vi "扫雷.vi"() -> ()   [LabVIEW 2017]
panel:
  out "上次索引":i32
  out "地图":u16[][](array[ring])
  out "游戏进行中":bool
  out "花费时间":dbl format="%<%M:%S>t"
  out "剩余地雷数":i32
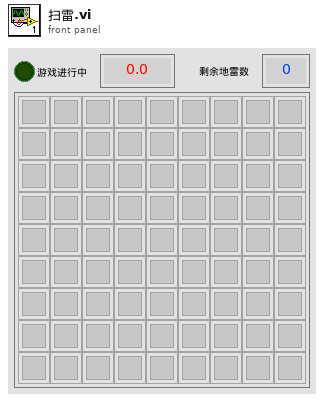
[diagram p1: front panel]
types:
  T1 = enum8{"Enabled", "Disabled", "Disabled and Grayed Out"}
  T2 = typedef "LVRectTypeDef.ctl" = cluster{"Left":i16, "Top":i16, "Right":i16, "Bottom":i16}
  T3 = typedef "LVBoundsTypeDef.ctl" = cluster{"Width":u32, "Height":u32}
  T4 = typedef "LVPositionTypeDef.ctl" = cluster{"Left":i32, "Top":i32}
  T5 = typedef "LVPoint32TypeDef.ctl" = cluster{"Horizontal":i32, "Vertical":i32}
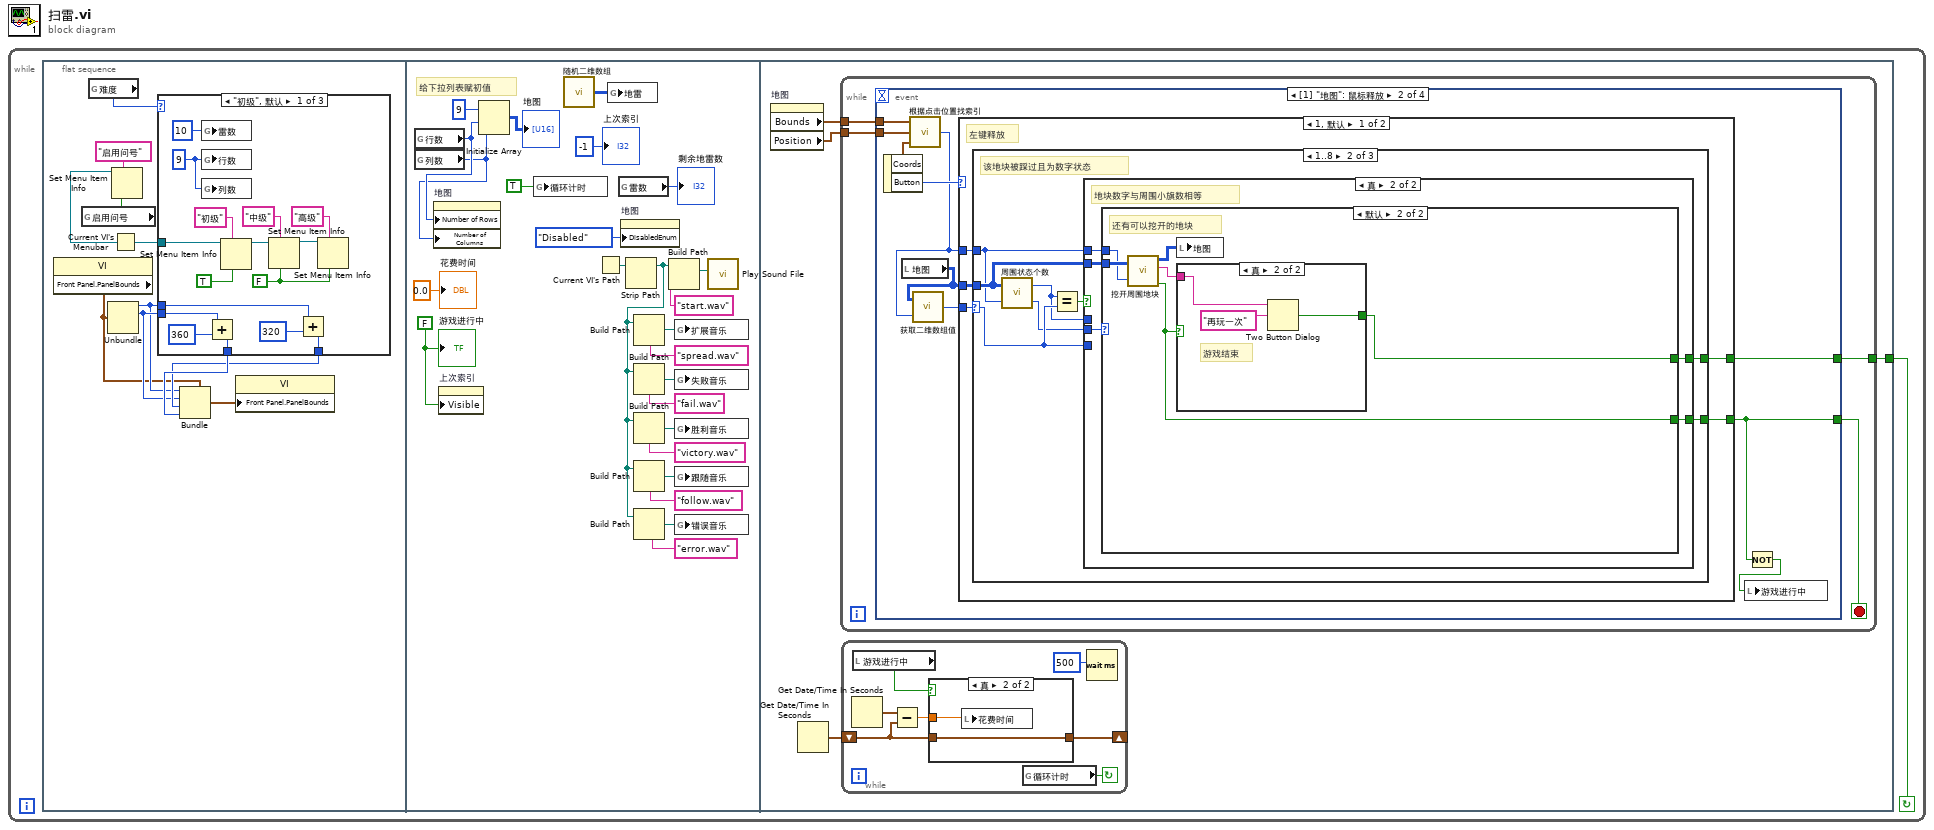
[diagram p0: block diagram]
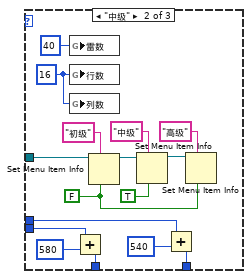
[diagram p2: hidden frame]
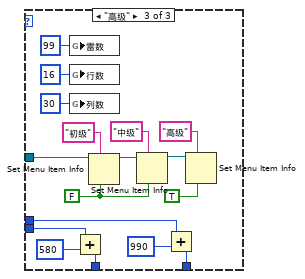
[diagram p3: hidden frame]
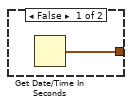
[diagram p4: hidden frame]
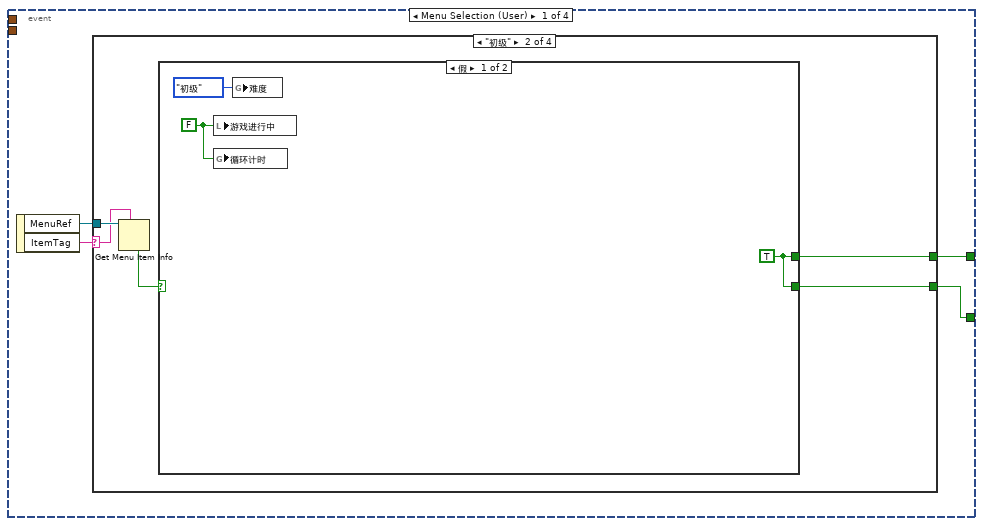
[diagram p5: hidden frame]
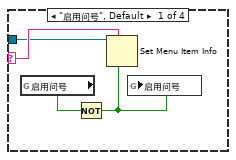
[diagram p6: hidden frame]
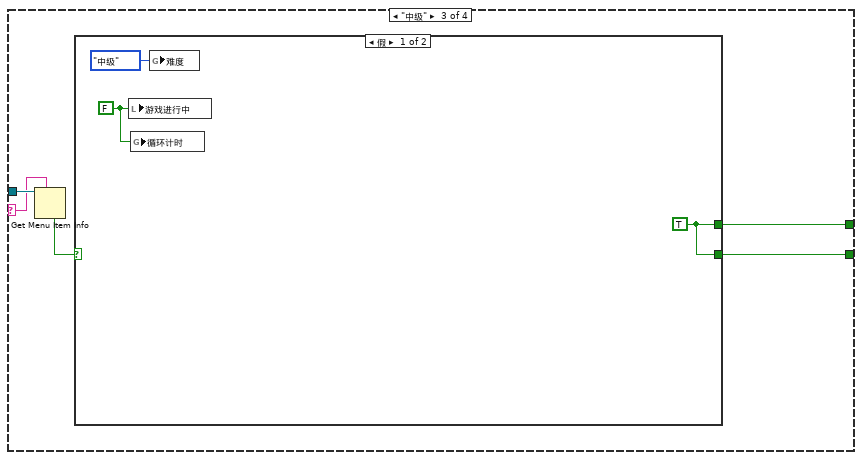
[diagram p8: hidden frame]
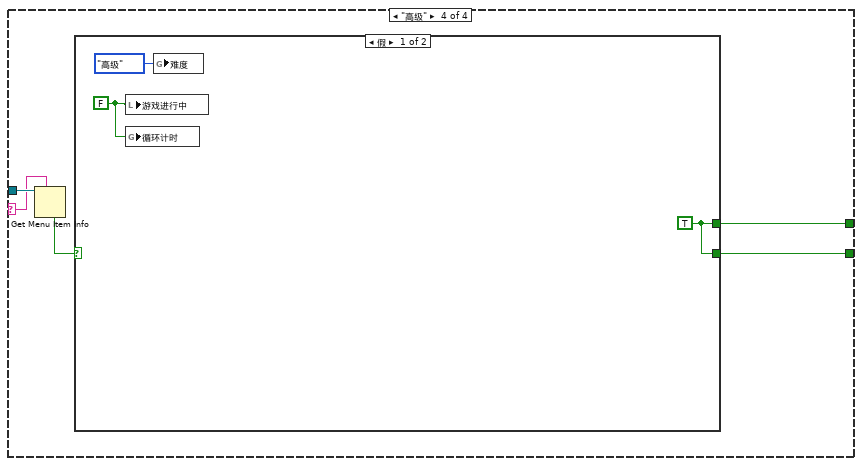
[diagram p10: hidden frame]
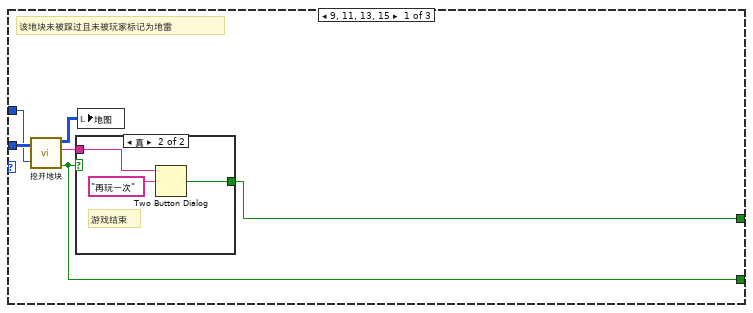
[diagram p12: hidden frame]
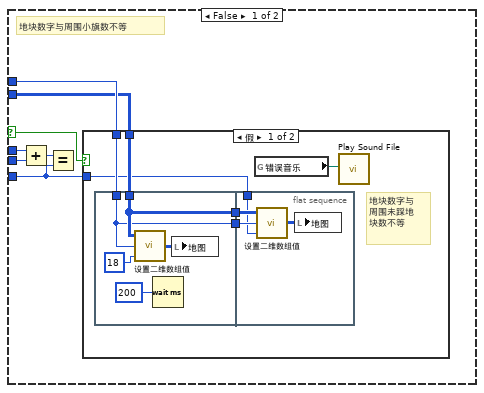
[diagram p14: hidden frame]
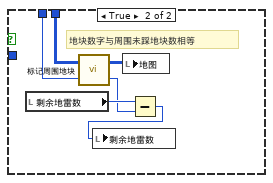
[diagram p15: hidden frame]
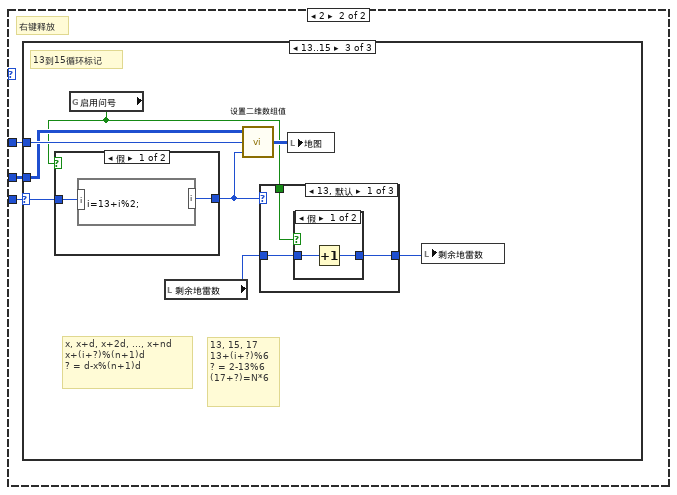
[diagram p19: hidden frame]
diagram:
  n1 = while {
    stop <- w1 continue-if-true
    n2 = flat-sequence {
      tunnel: [w89] -> w1
      frame #0 {
        n3 = property class="VI"() -> ("Front Panel.PanelBounds"=w2:T2)  [unwired: 2 in, 2 out]
        n4 = global read "全局变量.vi" "启用问号"() -> (w8:bool)
        n5 = global read "全局变量.vi" "难度"() -> (w11:enum16{"初级", "中级", "高级"})
        n6 = Unbundle(w2) -> ("Left"=w4:i16, "Top"=w5:i16)  [unwired: 2 out]
        n7 = Current VI's Menubar() -> (w9:refnum<k9>)
        n8 = Set Menu Item Info(6:w8, 7:"启用问号" ("项标识符"), 11:w9) -> ()  [unwired: 4 in, 2 out]
        n9 = case shown="\"初级\", 默认" w11 {
          tunnel: w9 -> [w18 w34 w50]
          tunnel: w4 -> [w17 w31 w47]
          tunnel: w5 -> [w16 w30 w46]
          tunnel: [w13 w28 w44] -> w6
          tunnel: [w15 w29 w45] -> w7
          frame "初级", Default {
            w19 = FALSE ("已勾选")
            w27 = i16 9 ("雷数")
            n10 = global write "全局变量.vi" "雷数"(i16 10 ("雷数")) -> ()
            n11 = global write "全局变量.vi" "行数"(w27) -> ()
            n12 = global write "全局变量.vi" "列数"(w27) -> ()
            n13 = Add(x=w16, y=i16 360) -> (x+y=w15:i16)
            n14 = Set Menu Item Info(6:TRUE ("已勾选"), 7:"初级" ("项标识符"), 11:w18) -> (3:w25:refnum<k9>)  [unwired: 4 in, 1 out]
            n15 = Set Menu Item Info(6:w19, 7:"中级" ("项标识符"), 11:w25) -> (3:w24:refnum<k9>)  [unwired: 4 in, 1 out]
            n16 = Add(x=w17, y=i16 320) -> (x+y=w13:i16)
            n17 = Set Menu Item Info(6:w19, 7:"高级" ("项标识符"), 11:w24) -> ()  [unwired: 4 in, 2 out]
          }
          frame "中级" {
            w35 = FALSE ("已勾选")
            w43 = i16 16 ("雷数")
            n18 = global write "全局变量.vi" "雷数"(i16 40 ("雷数")) -> ()
            n19 = global write "全局变量.vi" "行数"(w43) -> ()
            n20 = global write "全局变量.vi" "列数"(w43) -> ()
            n21 = Add(x=w30, y=i16 580) -> (x+y=w29:i16)
            n22 = Set Menu Item Info(6:w35, 7:"初级" ("项标识符"), 11:w34) -> (3:w41:refnum<k9>)  [unwired: 4 in, 1 out]
            n23 = Set Menu Item Info(6:TRUE ("已勾选"), 7:"中级" ("项标识符"), 11:w41) -> (3:w40:refnum<k9>)  [unwired: 4 in, 1 out]
            n24 = Add(x=w31, y=i16 540) -> (x+y=w28:i16)
            n25 = Set Menu Item Info(6:w35, 7:"高级" ("项标识符"), 11:w40) -> ()  [unwired: 4 in, 2 out]
          }
          frame "高级" {
            w51 = FALSE ("已勾选")
            n26 = global write "全局变量.vi" "雷数"(i16 99 ("雷数")) -> ()
            n27 = global write "全局变量.vi" "行数"(i16 16 ("雷数")) -> ()
            n28 = global write "全局变量.vi" "列数"(i16 30 ("列数")) -> ()
            n29 = Add(x=w46, y=i16 580) -> (x+y=w45:i16)
            n30 = Set Menu Item Info(6:w51, 7:"初级" ("项标识符"), 11:w50) -> (3:w57:refnum<k9>)  [unwired: 4 in, 1 out]
            n31 = Set Menu Item Info(6:w51, 7:"中级" ("项标识符"), 11:w57) -> (3:w56:refnum<k9>)  [unwired: 4 in, 1 out]
            n32 = Add(x=w47, y=i16 990) -> (x+y=w44:i16)
            n33 = Set Menu Item Info(6:TRUE ("已勾选"), 7:"高级" ("项标识符"), 11:w56) -> ()  [unwired: 4 in, 2 out]
          }
        }
        n34 = Bundle(cluster=w2, "Left"=w4, "Top"=w5, "Right"=w6, "Bottom"=w7) -> (w3:T2)
        n35 = property class="VI"("Front Panel.PanelBounds"=w3) -> ()  [unwired: 2 in, 2 out]
      }
      frame #1 {
        w72 = FALSE ("游戏进行中")
        # "给下拉列表赋初值"
        n36 = global read "全局变量.vi" "行数"() -> (w62:i32)
        n37 = global read "全局变量.vi" "列数"() -> (w61:i32)
        n38 = property on="地图" class="Arr (严格)"("Number of Rows"=w62, "Number of Columns"=w61) -> ()  [unwired: 2 in, 2 out]
        n39 = property on="上次索引" class="DigNum (严格)"("Visible"=w72) -> ()  [unwired: 2 in, 2 out]
        n40 = Initialize Array(9, w62, w61) -> (→"地图":i32[][])
        n41 = global write "全局变量.vi" "循环计时"(TRUE ("计时循环")) -> ()
        n42 = call "随机二维数组.vi"() -> ("数组"=w85:i16[][])
        n43 = Current VI's Path() -> (path=w81:path)
        n44 = global write "全局变量.vi" "地雷"(w85) -> ()
        n45 = global read "全局变量.vi" "雷数"() -> (→"剩余地雷数":i32)
        n46 = property on="地图" class="Arr (严格)"("DisabledEnum"=T1."Disabled" ("禁用")) -> ()  [unwired: 2 in, 2 out]
        n47 = Strip Path(path=w81) -> (stripped path=w74:path)  [unwired: 1 out]
        n48 = Build Path(base path=w74, name or relative path="spread.wav" ("名称或相对路径")) -> (appended path=w71:path)
        n49 = Build Path(base path=w74, name or relative path="fail.wav" ("名称或相对路径")) -> (appended path=w70:path)
        n50 = Build Path(base path=w74, name or relative path="victory.wav" ("名称或相对路径")) -> (appended path=w69:path)
        n51 = Build Path(base path=w74, name or relative path="follow.wav" ("名称或相对路径")) -> (appended path=w68:path)
        n52 = Build Path(base path=w74, name or relative path="error.wav" ("名称或相对路径")) -> (appended path=w67:path)
        n53 = Build Path(base path=w74, name or relative path="start.wav" ("名称或相对路径")) -> (appended path=w80:path)
        n54 = global write "全局变量.vi" "扩展音乐"(w71) -> ()
        n55 = global write "全局变量.vi" "失败音乐"(w70) -> ()
        n56 = global write "全局变量.vi" "胜利音乐"(w69) -> ()
        n57 = global write "全局变量.vi" "跟随音乐"(w68) -> ()
        n58 = global write "全局变量.vi" "错误音乐"(w67) -> ()
        n59 = call <vilib>:"Play Sound File.vi"("path"=w80) -> ()  [unwired: 9 in, 2 out]
        "游戏进行中" <- w72
        "花费时间" <- 0.0 ("花费时间")
        "上次索引" <- -1 ("上次索引")
      }
      frame #2 {
        n60 = property on="地图" class="Arr (严格)"() -> ("Bounds"=w87:T3, "Position"=w86:T4)  [unwired: 2 in, 2 out]
        n61 = Get Date/Time In Seconds() -> (seconds since 1Jan1904=w88:timestamp)
        n62 = while {
          tunnel: [w101] -> w89
          tunnel: w87 -> [w103]
          tunnel: w86 -> [w102]
          stop <- w100 stop-if-true
          n63 = event shown="[1] \"地图\": 鼠标释放" {
            selector: _ -> [_ _ _ _]
            dyn-events: _ -> [_ _ _ _]
            timeout: _ -> [_ _ _ _]
            tunnel: [w105 w141 _ _] -> w101
            tunnel: w103 -> [_ w145 w240 _]
            tunnel: w102 -> [_ w144 w239 _]
            tunnel: [w104 w140 _ _] -> w100
            event Menu Selection (User) {
              n64 = event-data() -> ("MenuRef"=w106:refnum<k9>, "ItemTag"=w107:string)  [unwired: 1 in]
              n65 = case shown="\"初级\"" w107 {
                selector: w107 -> [w111 w114 w122 w130]
                tunnel: w106 -> [w109 w116 w123 w131]
                tunnel: [_ w113 w121 w129] -> w105
                tunnel: [_ w112 w120 w128] -> w104
                frame "启用问号", Default {
                  n66 = global read "全局变量.vi" "启用问号"() -> (w110:bool)
                  n67 = Not(x=w110) -> (.not. x?=w108:bool)
                  n68 = Set Menu Item Info(6:w108, 7:w111, 11:w109) -> ()  [unwired: 4 in, 2 out]
                  n69 = global write "全局变量.vi" "启用问号"(w108) -> ()
                }
                frame "初级" {
                  n70 = Get Menu Item Info(7:w114, 11:w116) -> (4:w115:bool)  [unwired: 1 in, 6 out]
                  n71 = case shown="假" w115 {
                    tunnel: [w119 _] -> w113
                    tunnel: [w119 _] -> w112
                    frame False {
                      w118 = FALSE ("游戏进行中")
                      w119 = TRUE
                      n72 = local write "游戏进行中"(w118) -> ()
                      n73 = global write "全局变量.vi" "循环计时"(w118) -> ()
                      n74 = global write "全局变量.vi" "难度"(enum16{"初级", "中级", "高级"}."初级" ("难度")) -> ()
                    }
                    frame True {
                    }
                  }
                }
                frame "中级" {
                  n75 = Get Menu Item Info(7:w122, 11:w123) -> (4:w124:bool)  [unwired: 1 in, 6 out]
                  n76 = case shown="假" w124 {
                    tunnel: [w127 _] -> w121
                    tunnel: [w127 _] -> w120
                    frame False {
                      w125 = FALSE ("游戏进行中")
                      w127 = TRUE
                      n77 = local write "游戏进行中"(w125) -> ()
                      n78 = global write "全局变量.vi" "循环计时"(w125) -> ()
                      n79 = global write "全局变量.vi" "难度"(enum16{"初级", "中级", "高级"}."中级" ("难度")) -> ()
                    }
                    frame True {
                    }
                  }
                }
                frame "高级" {
                  n80 = Get Menu Item Info(7:w130, 11:w131) -> (4:w132:bool)  [unwired: 1 in, 6 out]
                  n81 = case shown="假" w132 {
                    tunnel: [w135 _] -> w129
                    tunnel: [w135 _] -> w128
                    frame False {
                      w133 = FALSE ("游戏进行中")
                      w135 = TRUE
                      n82 = local write "游戏进行中"(w133) -> ()
                      n83 = global write "全局变量.vi" "循环计时"(w133) -> ()
                      n84 = global write "全局变量.vi" "难度"(enum16{"初级", "中级", "高级"}."高级" ("难度")) -> ()
                    }
                    frame True {
                    }
                  }
                }
              }
            }
            event "地图": Mouse Up {
              n85 = event-data() -> ("Coords"=w143:T5, "Button"=w142:u16)  [unwired: 1 in]
              n86 = local read "地图"() -> (w137:u16[][])
              n87 = call "根据点击位置找索引.vi"("坐标"=w143, "位置"=w144, "边界"=w145) -> ("索引"=w138:i32)
              n88 = call "获取二维数组值.vi"("索引"=w138, "数组"=w137) -> ("数值"=w139:i32)
              n89 = case shown="1, 默认" w142 {
                tunnel: [w150 _] -> w141
                tunnel: [w149 _] -> w140
                tunnel: w139 -> [w148 w212]
                tunnel: w138 -> [w147 w211]
                tunnel: w137 -> [w146 w210]
                frame 1, Default {
                  # "左键释放"
                  n90 = case shown="1..8" w148 {
                    selector: w148 -> [_ w166 _]
                    tunnel: [w151 w161 _] -> w150
                    tunnel: [w153 w160 _] -> w149
                    tunnel: w147 -> [w155 w164 _]
                    tunnel: w146 -> [w156 w165 _]
                    frame 9, 11, 13, 15 {
                      # "该地块未被踩过且未被玩家标记为地雷"
                      n91 = call "挖开地块.vi"("地图"=w156, "索引"=w155) -> ("输出地图"=w154:i32[][], "对话框信息"=w152:string, "游戏结束"=w153:bool)  [unwired: 1 out]
                      n92 = case shown="真" w153 {
                        tunnel: w152 -> [_ w158]
                        tunnel: [_ w157] -> w151
                        frame False {
                        }
                        frame True {
                          # "游戏结束"
                          n93 = Two Button Dialog(message=w158, 2:"再玩一次" ("T按钮名称（“确定”）")) -> (T button?=w157:bool)  [unwired: 1 in]
                        }
                      }
                      n94 = local write "地图"(w154) -> ()
                    }
                    frame 1..8 {
                      # "该地块被踩过且为数字状态"
                      n95 = call "周围状态个数.vi"("索引"=w164, "地图"=w165) -> ("未标记数"=w162:i32, "标记数"=w163:i32)
                      n96 = Equal?(x=w163, y=w166) -> (x = y?=w167:bool)
                      n97 = case shown="真" w167 {
                        selector: w167 -> [w168 _]
                        tunnel: w165 -> [w172 w199]
                        tunnel: w164 -> [w173 w198]
                        tunnel: w166 -> [w171 _]
                        tunnel: w163 -> [w170 _]
                        tunnel: w162 -> [w169 w200]
                        tunnel: [_ w197] -> w161
                        tunnel: [_ w196] -> w160
                        frame False {
                          # "地块数字与周围小旗数不等"
                          n98 = Add(x=w170, y=w169) -> (x+y=w174:i32)
                          n99 = Equal?(x=w174, y=w171) -> ()  [unwired: 1 out]
                          n100 = case shown="假" w168 {
                            tunnel: w173 -> [w179 w195]
                            tunnel: w172 -> [w180 w194]
                            tunnel: w171 -> [w176 _]
                            frame False {
                              # "地块数字与\n周围未踩地\n块数不等"
                              n101 = flat-sequence {
                                tunnel: w180 -> [w183]
                                tunnel: w179 -> [w182]
                                tunnel: [w183] -> w178
                                tunnel: [w182] -> w177
                                tunnel: w178 -> [w189]
                                tunnel: w177 -> [w188]
                                tunnel: w176 -> [w187]
                                frame #0 {
                                n102 = call "设置二维数组值.vi"("数值"=18, "索引"=w182, "数组"=w183) -> ("输出数组"=w184:i32[][])
                                n103 = Wait (ms)(milliseconds to wait=u32 200 ("毫秒倍数")) -> ()  [unwired: 1 out]
                                n104 = local write "地图"(w184) -> ()
                                }
                                frame #1 {
                                n105 = call "设置二维数组值.vi"("数值"=w187, "索引"=w188, "数组"=w189) -> ("输出数组"=w186:i32[][])
                                n106 = local write "地图"(w186) -> ()
                                }
                              }
                              n107 = global read "全局变量.vi" "错误音乐"() -> (w175:path)
                              n108 = call <vilib>:"Play Sound File.vi"("path"=w175) -> ()  [unwired: 9 in, 2 out]
                            }
                            frame True {
                              # "地块数字与周围未踩地块数相等"
                              n109 = local read "剩余地雷数"() -> (w192:i32)
                              n110 = call "标记周围地块.vi"("索引"=w195, "地图"=w194) -> ("标记个数"=w191:i32, "输出地图"=w193:i32[][])
                              n111 = local write "地图"(w193) -> ()
                              n112 = Subtract(x=w192, y=w191) -> (x-y=w190:i32)
                              n113 = local write "剩余地雷数"(w190) -> ()
                            }
                          }
                        }
                        frame True {
                          # "地块数字与周围小旗数相等"
                          n114 = case shown="默认" w200 {
                            tunnel: w199 -> [_ w206]
                            tunnel: w198 -> [_ w205]
                            tunnel: [_ w202] -> w197
                            tunnel: [_ w201] -> w196
                            frame 0 {
                              # "没有可以挖开的地块"
                            }
                            frame Default {
                              # "还有可以挖开的地块"
                              n115 = call "挖开周围地块.vi"("地图"=w206, "索引"=w205) -> ("输出地图"=w204:i32[][], "对话框信息"=w203:string, "游戏结束"=w201:bool)  [unwired: 1 out]
                              n116 = local write "地图"(w204) -> ()
                              n117 = case shown="真" w201 {
                                tunnel: w203 -> [_ w208]
                                tunnel: [_ w207] -> w202
                                frame False {
                                }
                                frame True {
                                # "游戏结束"
                                n118 = Two Button Dialog(message=w208, 2:"再玩一次" ("T按钮名称（“确定”）")) -> (T button?=w207:bool)  [unwired: 1 in]
                                }
                              }
                            }
                          }
                        }
                      }
                    }
                    frame 10, 14, Default {
                      # "该地块被玩家标记为地雷"
                    }
                  }
                }
                frame 2 {
                  # "右键释放"
                  n119 = case shown="13..15" w212 {
                    selector: w212 -> [_ _ w218]
                    tunnel: w211 -> [_ _ w220]
                    tunnel: w210 -> [_ _ w214]
                    frame Default {
                      # "无响应"
                    }
                    frame 1..8 {
                      # "地块为数字状态"
                    }
                    frame 13..15 {
                      # "13, 15, 17\n13+(i+?)%6\n? = 2-13%6\n(17+?)=N*6"
                      # "x, x+d, x+2d, ..., x+nd\nx+(i+?)%(n+1)d\n? = d-x%(n+1)d"
                      # "13到15循环标记"
                      n120 = global read "全局变量.vi" "启用问号"() -> (w213:bool)
                      n121 = case shown="假" w213 {
                        tunnel: w218 -> [w222 w224]
                        tunnel: [w221 w223] -> w217
                        frame False {
                          n122 = formula code="i=13+i%2;"("i"=w222) -> ("i"=w221:i32)
                        }
                        frame True {
                          n123 = formula code="i=13+i%3;"("i"=w224) -> ("i"=w223:i32)
                        }
                      }
                      n124 = local read "剩余地雷数"() -> (w215:i32)
                      n125 = call "设置二维数组值.vi"("数值"=w217, "索引"=w220, "数组"=w214) -> ("输出数组"=w219:i32[][])
                      n126 = case shown="13, 默认" w217 {
                        tunnel: [w226 w231 w233] -> w216
                        tunnel: w215 -> [w227 w232 w234]
                        tunnel: w213 -> [w225 _ _]
                        frame 13, Default {
                          n127 = case shown="假" w225 {
                            tunnel: w227 -> [w229 w230]
                            tunnel: [w228 w230] -> w226
                            frame False {
                              n128 = Increment(x=w229) -> (x+1=w228:i32)
                            }
                            frame True {
                            }
                          }
                        }
                        frame 14 {
                          n129 = Decrement(x=w232) -> (x-1=w231:i32)
                        }
                        frame 15 {
                          n130 = Increment(x=w234) -> (x+1=w233:i32)
                        }
                      }
                      n131 = local write "地图"(w219) -> ()
                      n132 = local write "剩余地雷数"(w216) -> ()
                    }
                  }
                }
              }
              n133 = Not(x=w140) -> (.not. x?=w136:bool)
              n134 = local write "游戏进行中"(w136) -> ()
            }
            event "地图": Mouse Move {
              n135 = event-data() -> ("Coords"=w238:T5)  [unwired: 1 in]
              n136 = call "根据点击位置找索引.vi"("坐标"=w238, "位置"=w239, "边界"=w240) -> ("索引"=w235:i32)
              n137 = local read "地图"() -> (w236:u16[][])
              n138 = call "获取二维数组值.vi"("索引"=w235, "数组"=w236) -> ("数值"=w237:i32)
              n139 = case shown="9..11" w237 {
                selector: w237 -> [_ w255 _]
                tunnel: w236 -> [w241 w256 _]
                tunnel: w235 -> [_ w254 _]
                frame 0..8 {
                  # "当前地块为数字状态"
                  n140 = local read "上次索引"() -> (w242:i32)
                  n141 = case shown="0, 默认" w242 {
                    selector: w242 -> [_ w244]
                    tunnel: w241 -> [_ w243]
                    frame -1 {
                    }
                    frame 0, Default {
                      n142 = call "获取二维数组值.vi"("索引"=w244, "数组"=w243) -> ("数值"=w245:i32)
                      n143 = case shown="13..15" w245 {
                        selector: w245 -> [_ w250]
                        tunnel: w244 -> [_ w252]
                        tunnel: w243 -> [_ w251]
                        frame 0, Default {
                        }
                        frame 13..15 {
                          n144 = Subtract(x=w250, y=4) -> (x-y=w249:i32)
                          n145 = call "设置二维数组值.vi"("数值"=w249, "索引"=w252, "数组"=w251) -> ("输出数组"=w247:i32[][])
                          n146 = local write "上次索引"(-1 ("上次索引")) -> ()
                          n147 = local write "地图"(w247) -> ()
                        }
                      }
                    }
                  }
                }
                frame 9..11 {
                  # "当前地块为初始状态"
                  n148 = flat-sequence {
                    tunnel: w256 -> [w265]
                    tunnel: w255 -> [w264]
                    tunnel: w254 -> [w258]
                    tunnel: [w258] -> w253
                    tunnel: w253 -> [w278]
                    frame #0 {
                      n149 = local read "上次索引"() -> (w259:i32)
                      n150 = Add(x=w264, y=4) -> (x+y=w263:i32)
                      n151 = call "设置二维数组值.vi"("数值"=w263, "索引"=w258, "数组"=w265) -> ("输出数组"=w261:i32[][])
                      n152 = case shown="0, 默认" w259 {
                        selector: w259 -> [_ w269]
                        tunnel: w261 -> [w266 w270]
                        tunnel: [w266 w268] -> w260
                        frame -1 {
                        }
                        frame 0, Default {
                          n153 = call "获取二维数组值.vi"("索引"=w269, "数组"=w270) -> ("数值"=w267:i32)
                          n154 = case shown="13..15" w267 {
                            selector: w267 -> [_ w272]
                            tunnel: w270 -> [w271 w275]
                            tunnel: w269 -> [_ w274]
                            tunnel: [w271 w273] -> w268
                            frame 0, Default {
                            }
                            frame 13..15 {
                              n155 = Subtract(x=w272, y=4) -> (x-y=w276:i32)
                              n156 = call "设置二维数组值.vi"("数值"=w276, "索引"=w274, "数组"=w275) -> ("输出数组"=w273:i32[][])
                            }
                          }
                        }
                      }
                      n157 = global read "全局变量.vi" "跟随音乐"() -> (w257:path)
                      n158 = call <vilib>:"Play Sound File.vi"("path"=w257) -> ()  [unwired: 9 in, 2 out]
                      n159 = local write "地图"(w260) -> ()
                    }
                    frame #1 {
                      n160 = local write "上次索引"(w278) -> ()
                    }
                  }
                }
                frame 13..15, Default {
                  # "当前地块为鼠标跟随状态"
                }
              }
            }
            event "地图": Mouse Leave {
              n161 = event-data() -> ()  [unwired: 1 in, 4 out]
              n162 = local read "上次索引"() -> (w279:i32)
              n163 = case shown="0, 默认" w279 {
                selector: w279 -> [_ w281]
                frame -1 {
                }
                frame 0, Default {
                  n164 = local read "地图"() -> (w280:u16[][])
                  n165 = call "获取二维数组值.vi"("索引"=w281, "数组"=w280) -> ("数值"=w282:i32)
                  n166 = case shown="13..15" w282 {
                    selector: w282 -> [_ w287]
                    tunnel: w281 -> [_ w289]
                    tunnel: w280 -> [_ w288]
                    frame 0, Default {
                    }
                    frame 13..15 {
                      n167 = Subtract(x=w287, y=4) -> (x-y=w286:i32)
                      n168 = call "设置二维数组值.vi"("数值"=w286, "索引"=w289, "数组"=w288) -> ("输出数组"=w284:i32[][])
                      n169 = local write "上次索引"(-1 ("上次索引")) -> ()
                      n170 = local write "地图"(w284) -> ()
                    }
                  }
                }
              }
            }
          }
        }
        n171 = while {
          shift-right: [w92] -> _
          shift-left: w88 -> [w91]
          stop <- w90 continue-if-true
          n172 = Get Date/Time In Seconds() -> (seconds since 1Jan1904=w96:timestamp)
          n173 = local read "游戏进行中"() -> (w93:bool)
          n174 = Subtract(x=w96, y=w91) -> (x-y=w95:dbl)
          n175 = case shown="真" w93 {
            tunnel: w95 -> [_ w99]
            tunnel: [w97 w98] -> w92
            tunnel: w91 -> [_ w98]
            frame False {
              n176 = Get Date/Time In Seconds() -> (seconds since 1Jan1904=w97:timestamp)
            }
            frame True {
              n177 = local write "花费时间"(w99) -> ()
            }
          }
          n178 = global read "全局变量.vi" "循环计时"() -> (w90:bool)
          n179 = Wait (ms)(milliseconds to wait=500) -> ()  [unwired: 1 out]
        }
      }
    }
  }
